vi "ccd.vi"() -> ()   [LabVIEW 2015]
panel:
  in  "Constante de condition\n(Voir l'aide contextuelle)":bool
  in  "trigEventString":string
  in  "trigSigTypeString":string
  in  "trigAddress":i32
  in  "Commande tab":enum32{"Settings", "Trigger In", "Infos"}(tab)
  in  "Integration time (ms) :":i16=10
  in  "Number of Areas :":u16=1 min=1 step=1
  in  "ADC":u16(ring) caption="Device Name" items=["20 kHz       ", " 1 MHz       ", "500 kHz Wrap"]
  in  "GAIN":u16(ring) caption="Device Name" items=["High Light", "Best Dynamic Range", "High Sensitivity"]
  in  "Device Name":u16(ring) items=["Synapse"]
  out "Uniques ID":u16(ring) items=["CCD1"]
  in  "Reformat":bool
  in  "Signal type :":enum16{"TTL Rising Edge", "TTL Falling Edge"}(ring)=enum."TTL Falling Edge"
  in  "Trigger Type :":enum16{"On Start", "Per Acquisition"}(ring)
  in  "Enable InputTriggers :":bool
  out "DataSize":i32=262144
  out "Y Pixels:":i32=256
  out "X Pixels:":i32=1024
  out "Firmware\nVersion":string="V1.20 CCD_4000"
  out "Acq Time(ms)":u32=2010
  out "ADC Number":i32[](array[numeric])=[0, 1, 2, 3, 4]
  out "Gain Number":i32[](array[numeric])=[10, 11, 12, 13, 8, 2]
  out "Intensity Graph":dbl[][](graph)
  in  "save":bool
  out "initialized ?":bool
  in  "Continuous":bool
  in  "CCD Busy":bool
  in  "Shutter Enable":bool=TRUE
  out "temp graph":dbl(graph)=66.11766439999997
  in  "Temperature":bool
  out "areas :":i32[][](array[numeric])=[[1], [1], [1], [1024], [256], [1], [1]]
  in  "Acquire":bool
  in  "Setup":bool
  in  "Close":bool=TRUE
  out "indicator":string
  in  "initialize":bool
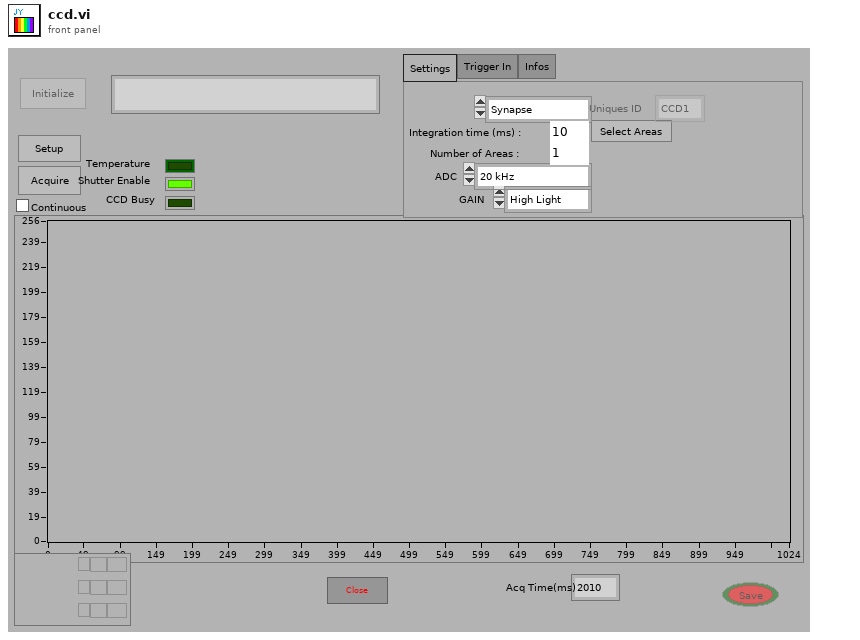
[diagram p1: front panel]
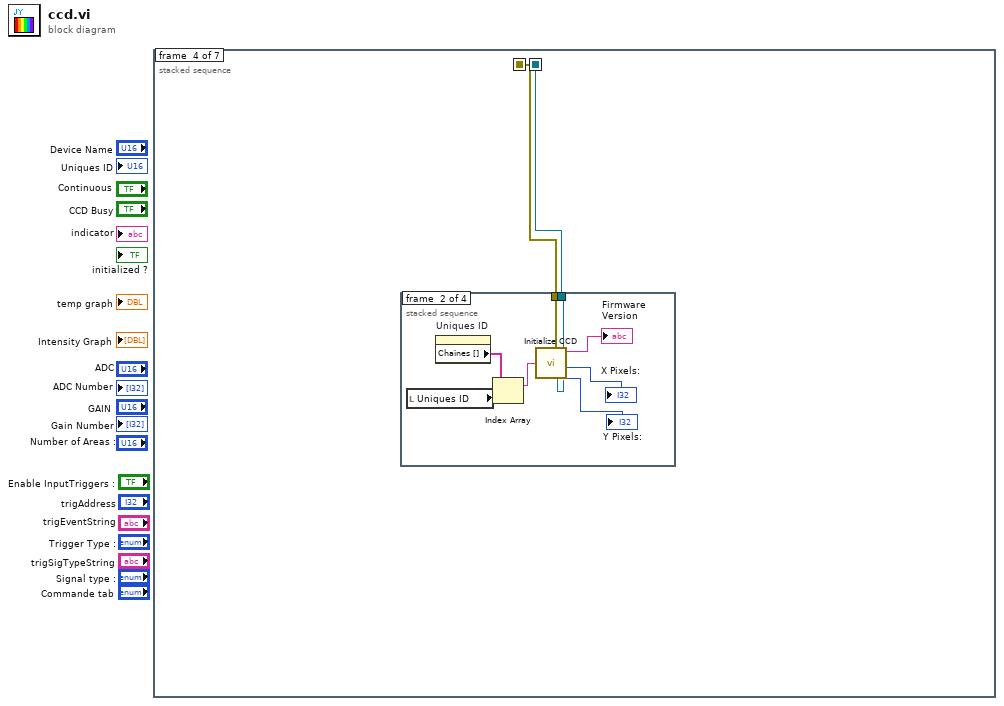
[diagram p0: block diagram]
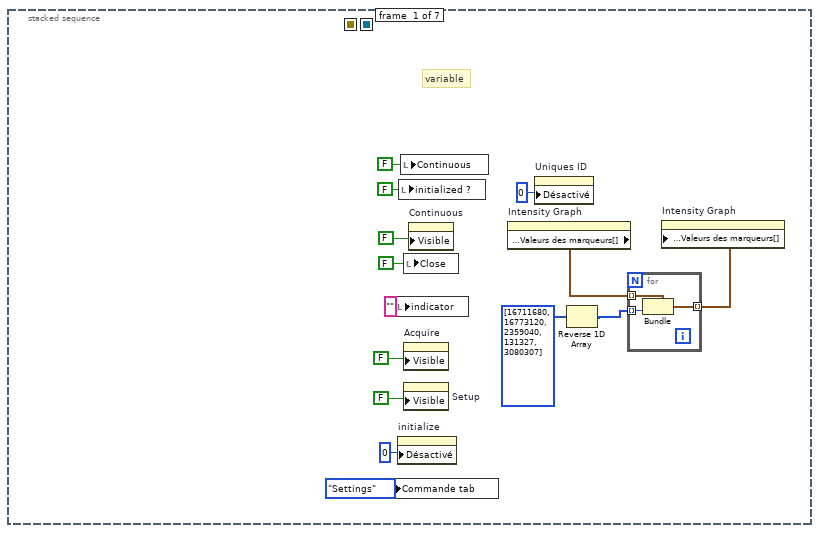
[diagram p2: hidden frame]
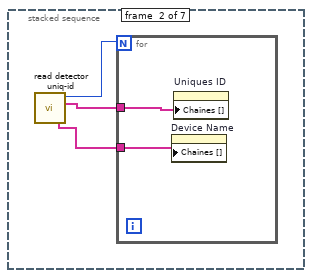
[diagram p3: hidden frame]
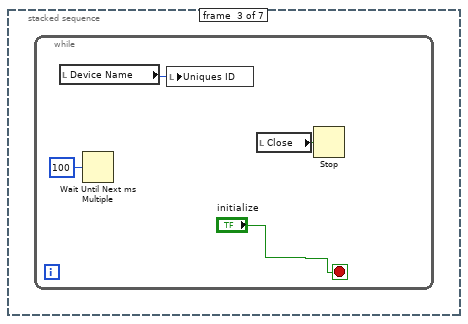
[diagram p4: hidden frame]
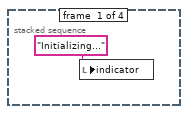
[diagram p5: hidden frame]
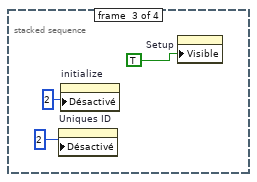
[diagram p6: hidden frame]
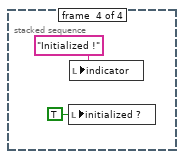
[diagram p7: hidden frame]
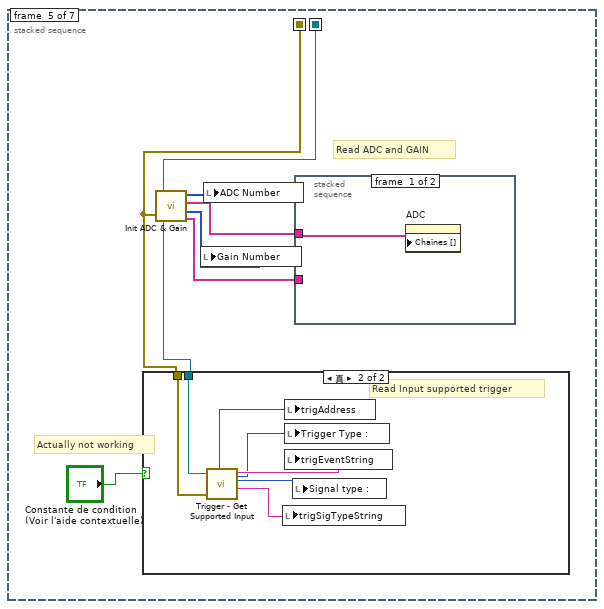
[diagram p8: hidden frame]
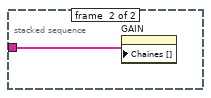
[diagram p10: hidden frame]
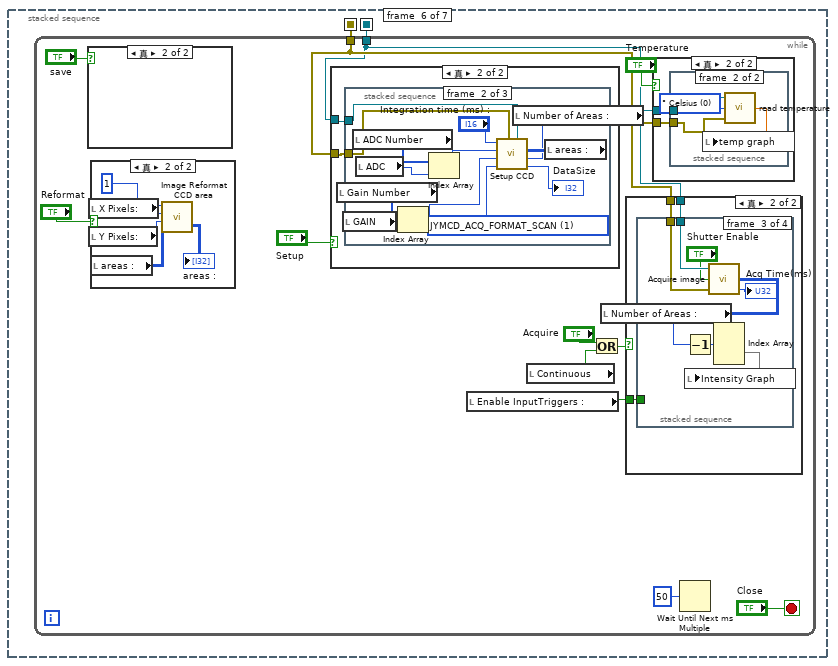
[diagram p11: hidden frame]
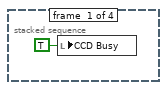
[diagram p14: hidden frame]
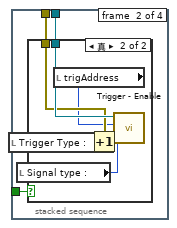
[diagram p15: hidden frame]
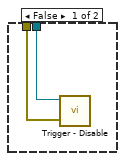
[diagram p16: hidden frame]
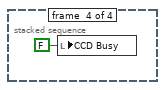
[diagram p17: hidden frame]
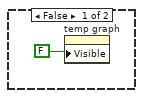
[diagram p18: hidden frame]
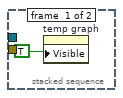
[diagram p19: hidden frame]
diagram:
  n1 = stacked-sequence {
    seq-local: [_ _ _ w28 _ _ _] -> [_ _ _ _ w44 w60 w128]
    seq-local: [_ _ _ w27 _ _ _] -> [_ _ _ _ w43 w59 w129]
    frame #0 {
      # "variable"
      n2 = local write "Commande tab"(enum32{"Settings", "Trigger In", "Infos"}."Settings" ("Commande tab")) -> ()
      n3 = local write "indicator"("" ("indicator")) -> ()
      n4 = property on="initialize" class="Bool"("Désactivé"=u8 0) -> ()  [unwired: 2 in, 2 out]
      n5 = local write "initialized ?"(FALSE ("initialized ?")) -> ()
      n6 = local write "Continuous"(FALSE ("Continuous")) -> ()
      n7 = local write "Close"(FALSE ("Close")) -> ()
      n8 = property on="Acquire" class="Bool"("Visible"=FALSE) -> ()  [unwired: 2 in, 2 out]
      n9 = property on="Setup" class="Bool"("Visible"=FALSE) -> ()  [unwired: 2 in, 2 out]
      n10 = property on="Continuous" class="Bool (严格)"("Visible"=FALSE) -> ()  [unwired: 2 in, 2 out]
      n11 = property on="Intensity Graph" class="IntGraph (严格)"() -> ("Échelle des Z.Valeurs des marqueurs[]"=w4:cluster{dbl, u32}[])  [unwired: 2 in, 2 out]
      n12 = property on="Uniques ID" class="Ring (严格)"("Désactivé"=u8 0) -> ()  [unwired: 2 in, 2 out]
      n13 = Reverse 1D Array(array=u32[] [16711680, 16773120, 2359040, 131327, 3080307] ("Sous-tableau")) -> (reversed array=w5:u32[])
      n14 = for {
        tunnel: w5 -> [w17] mode=indexing
        tunnel: [w16] -> w3 mode=indexing
        tunnel: w4 -> [w15] mode=indexing
        n15 = Bundle(cluster=w15, w17) -> (w16:cluster{dbl, u32})  [unwired: 1 out]
      }
      n16 = property on="Intensity Graph" class="IntGraph (严格)"("Échelle des Z.Valeurs des marqueurs[]"=w3) -> ()  [unwired: 2 in, 2 out]
    }
    frame #1 {
      n17 = call <userlib>:"read detector uniq-id.vi"() -> ("nbr of components"=w20:i32, "UniqueID"=w19:string[], "Name"=w18:string[])  [unwired: 4 out]
      n18 = for {
        N: w20 -> [_]
        tunnel: w19 -> [w22]
        tunnel: w18 -> [w21]
        n19 = property on="Device Name" class="Ring (严格)"("Chaînes []"=w21) -> ()  [unwired: 2 in, 2 out]
        n20 = property on="Uniques ID" class="Ring (严格)"("Chaînes []"=w22) -> ()  [unwired: 2 in, 2 out]
      }
    }
    frame #2 {
      n21 = while {
        stop <- "initialize" stop-if-true
        n22 = local read "Device Name"() -> (w25:u16)
        n23 = Wait Until Next ms Multiple(millisecond multiple=u32 100 ("n millisecondes")) -> ()  [unwired: 1 out]
        n24 = local write "Uniques ID"(w25) -> ()
        n25 = local read "Close"() -> (w23:bool)
        n26 = Stop(stop? (T)=w23) -> ()
      }
    }
    frame #3 {
      n27 = stacked-sequence {
        tunnel: [_ w34 _ _] -> w28
        tunnel: [_ w33 _ _] -> w27
        frame #0 {
          n28 = local write "indicator"("Initializing..." ("indicator")) -> ()
        }
        frame #1 {
          n29 = local read "Uniques ID"() -> (w31:u16)
          n30 = property on="Uniques ID" class="Ring (严格)"() -> ("Chaînes []"=w32:string[])  [unwired: 2 in, 2 out]
          n31 = Index Array(array=w32, index=w31) -> (element=w30:string)
          n32 = call <userlib>:"Initialize CCD.vi"("Unique id:"=w30) -> ("activeYPixels"=→"Y Pixels:":i32, "JYCCDLib.IJYCCDReqd"=w33:refnum<k7>, "activeXPixels"=→"X Pixels:":i32, "sortie d'erreur"=w34:errorcluster, "FirmwareVersion"=→"Firmware\nVersion":string)  [unwired: 3 out]
        }
        frame #2 {
          n33 = property on="Uniques ID" class="Ring (严格)"("Désactivé"=u8 2) -> ()  [unwired: 2 in, 2 out]
          n34 = property on="initialize" class="Bool"("Désactivé"=u8 2) -> ()  [unwired: 2 in, 2 out]
          n35 = property on="Setup" class="Bool"("Visible"=TRUE) -> ()  [unwired: 2 in, 2 out]
        }
        frame #3 {
          n36 = local write "initialized ?"(TRUE ("initialized ?")) -> ()
          n37 = local write "indicator"("Initialized !" ("indicator")) -> ()
        }
      }
    }
    frame #4 {
      # "Actually not working"
      # "Read ADC and GAIN"
      n38 = case shown="真" "Constante de condition\n(Voir l'aide contextuelle)" {
        tunnel: w43 -> [_ w56]
        tunnel: w44 -> [_ w55]
        frame False {
        }
        frame True {
          # "Read Input supported trigger"
          n39 = call <userlib>:"Trigger - Get Supported Input.vi"("JYCCDLib.IJYCCDReqd"=w56, "Error Input"=w55) -> ("trigAddress"=w50:i32, "eventPtr"=w51:i32, "trigEventString"=w54:string, "trigSigType"=w53:i32, "trigSigTypeString"=w52:string)  [unwired: 4 out]
          n40 = local write "trigSigTypeString"(w52) -> ()
          n41 = local write "trigAddress"(w50) -> ()
          n42 = local write "Trigger Type :"(w51) -> ()
          n43 = local write "trigEventString"(w54) -> ()
          n44 = local write "Signal type :"(w53) -> ()
        }
      }
      n45 = call <userlib>:"Init ADC & Gain.vi"("JYCCDLib.IJYCCDReqd"=w43, "input error"=w44) -> ("ADC Number"=w47:i32[], "ADC description"=w49:string[], "Gain Number"=w46:i32[], "Gain description"=w48:string[])
      n46 = local write "Gain Number"(w46) -> ()
      n47 = local write "ADC Number"(w47) -> ()
      n48 = stacked-sequence {
        tunnel: w49 -> [w57 _]
        tunnel: w48 -> [_ w58]
        frame #0 {
          n49 = property on="ADC" class="Ring (严格)"("Chaînes []"=w57) -> ()  [unwired: 2 in, 2 out]
        }
        frame #1 {
          n50 = property on="GAIN" class="Ring (严格)"("Chaînes []"=w58) -> ()  [unwired: 2 in, 2 out]
        }
      }
    }
    frame #5 {
      n51 = while {
        tunnel: w59 -> [w62]
        tunnel: w60 -> [w64]
        stop <- "Close" stop-if-true
        n52 = case shown="真" "save" {
          frame False {
          }
          frame True {
          }
        }
        n53 = case shown="真" "Reformat" {
          frame False {
          }
          frame True {
            n54 = local read "X Pixels:"() -> (w107:i32)
            n55 = local read "Y Pixels:"() -> (w109:i32)
            n56 = local read "areas :"() -> (w105:i32[][])
            n57 = call <userlib>:"Image Reformat CCD area.vi"("areas :"=w105, "Y Pixels:"=w109, "X Pixels:"=w107, "numAreas"=1) -> ("areas"=→"areas :":i32[][])  [unwired: 1 out]
          }
        }
        n58 = case shown="真" "Setup" {
          tunnel: w64 -> [_ w110]
          tunnel: w62 -> [_ w111]
          frame False {
          }
          frame True {
            n59 = stacked-sequence {
              tunnel: w110 -> [_ w125 _]
              tunnel: w111 -> [_ w122 _]
              frame #0 {
                n60 = local write "indicator"("Setting up the detector" ("indicator")) -> ()
              }
              frame #1 {
                w123 = 1 items=["JYMCD_ACQ_FORMAT_IMAGE", "JYMCD_ACQ_FORMAT_SCAN"] ("Acquisition type")
                n61 = local read "Gain Number"() -> (w117:i32[])
                n62 = local read "GAIN"() -> (w113:u16)
                n63 = local read "ADC Number"() -> (w118:i32[])
                n64 = local read "ADC"() -> (w114:u16)
                n65 = Index Array(array=w117, index=w113) -> (element=w115:i32)
                n66 = Index Array(array=w118, index=w114) -> (element=w116:i32)
                n67 = local read "Number of Areas :"() -> (w120:u16)
                n68 = local read "areas :"() -> (w121:i32[][])
                n69 = call <userlib>:"Setup CCD.vi"("numAreas"=w120, "areas :"=w121, "JYCCDLib.IJYCCDReqd"=w122, "entrée d'erreur (pas d'erreur)"=w125, "Acquisition type"=w123, "Gain"=w115, "Select ADC"=w116, "Integration time(ms)"="Integration time (ms) :") -> ("DataSize"=→"DataSize":i32)  [unwired: 1 out]
              }
              frame #2 {
                w126 = TRUE ("Visible")
                n70 = property on="Acquire" class="Bool"("Visible"=w126) -> ()  [unwired: 2 in, 2 out]
                n71 = local write "indicator"("Ready !" ("indicator")) -> ()
                n72 = property on="Continuous" class="Bool (严格)"("Visible"=w126) -> ()  [unwired: 2 in, 2 out]
              }
            }
          }
        }
        n73 = local read "Enable InputTriggers :"() -> (w61:bool)
        n74 = local read "Continuous"() -> (w65:bool)
        n75 = Or(x="Acquire", y=w65) -> (x .or. y?=w67:bool)
        n76 = case shown="真" w67 {
          tunnel: w62 -> [_ w75]
          tunnel: w64 -> [_ w74]
          tunnel: w61 -> [_ w73]
          frame False {
          }
          frame True {
            n77 = stacked-sequence {
              tunnel: w75 -> [_ w78 w95 _]
              tunnel: w74 -> [_ w77 w94 _]
              tunnel: w73 -> [_ w79 _ _]
              frame #0 {
                n78 = local write "CCD Busy"(TRUE ("CCD Busy")) -> ()
              }
              frame #1 {
                n79 = case shown="真" w79 {
                  tunnel: w78 -> [w81 w87]
                  tunnel: w77 -> [w80 w86]
                  frame False {
                    n80 = call <userlib>:"Trigger - Disable.vi"("Error In"=w80, "JYCCDLib.IJYCCDReqd"=w81) -> ()  [unwired: 6 out]
                  }
                  frame True {
                    n81 = local read "Trigger Type :"() -> (w84:enum16{"On Start", "Per Acquisition"})
                    n82 = local read "Signal type :"() -> (w83:enum16{"TTL Rising Edge", "TTL Falling Edge"})
                    n83 = local read "trigAddress"() -> (w85:i32)
                    n84 = Increment(x=w84) -> (x+1=w82:enum16{"On Start", "Per Acquisition"})
                    n85 = call <userlib>:"Trigger - Enable.vi"("Error In"=w86, "sigType"=w83, "event"=w82, "trigAddress"=w85, "JYCCDLib.IJYCCDReqd"=w87) -> ()  [unwired: 3 out]
                  }
                }
              }
              frame #2 {
                n86 = local read "Number of Areas :"() -> (w89:u16)
                n87 = Decrement(x=w89) -> (x-1=w91:u16)
                n88 = call <userlib>:"Acquire image.vi"("error in"=w94, "ShutterOpen"="Shutter Enable", "JYCCDLib.IJYCCDReqd"=w95) -> ("Acq Time(ms)"=→"Acq Time(ms)":u32, "Datas"=w92:i32[][][])  [unwired: 1 out]
                n89 = Index Array(array=w92, index (dim 0)=w91) -> (element=w90:i32[][])  [unwired: 2 in]
                n90 = local write "Intensity Graph"(w90) -> ()
              }
              frame #3 {
                n91 = local write "CCD Busy"(FALSE ("CCD Busy")) -> ()
              }
            }
          }
        }
        n92 = case shown="真" "Temperature" {
          tunnel: w62 -> [_ w99]
          tunnel: w64 -> [_ w98]
          frame False {
            n93 = property on="temp graph" class="WFChart (严格)"("Visible"=FALSE) -> ()  [unwired: 2 in, 2 out]
          }
          frame True {
            n94 = stacked-sequence {
              tunnel: w99 -> [_ w104]
              tunnel: w98 -> [_ w103]
              frame #0 {
                n95 = property on="temp graph" class="WFChart (严格)"("Visible"=TRUE) -> ()  [unwired: 2 in, 2 out]
              }
              frame #1 {
                w102 = u16 0 items=["° Celsius", "Kelvin", "° Farenheit"] ("units")
                n96 = call <userlib>:"read temperature.vi"("entrée d'erreur (pas d'erreur)"=w103, "units"=w102, "JYCCDLib.IJYCCDReqd"=w104) -> ("Current Temperature"=w101:dbl)
                n97 = local write "temp graph"(w101) -> ()
              }
            }
          }
        }
        n98 = Wait Until Next ms Multiple(millisecond multiple=u32 50 ("n millisecondes")) -> ()  [unwired: 1 out]
      }
    }
    frame #6 {
      n99 = Close Reference(reference=w129, error in (no error)=w128) -> ()  [unwired: 1 out]
    }
  }
